vi "Update Bind Method Constants.vi"(7 "RPC Method Parameters":T1, 8 "error in (no error)":errorcluster, 10 "RPC Method Name":string, 11 "VI in":refnum<vi>) -> (0 "error out":errorcluster, 3 "VI out":refnum<vi>)   [LabVIEW 2019, in "gRPC Template Creation Utility.lvlib"]
uses:
  gRPC Template Creation Utility.lvlib
  TypeDefs/RPC Method Parameters.ctl
  <vilib>/Utility/traverseref.llb/TRef TravTarget.ctl
  <vilib>/Utility/traverseref.llb/VI Scripting - Traverse.lvlib
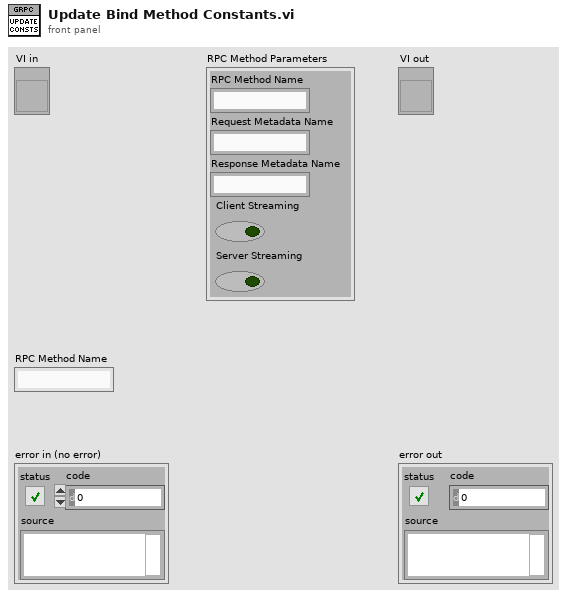
[diagram p1: front panel]
types:
  T1 = typedef "gRPC Template Creation Utility.lvlib/RPC Method Parameters.ctl" = cluster{"RPC Method Name":string, "Request Metadata Name":string, "Response Metadata Name":string, "Client Streaming":bool, "Server Streaming":bool}
  T2 = typedef "TRef TravTarget.ctl" = enum16{"FP", "BD", "Other"}
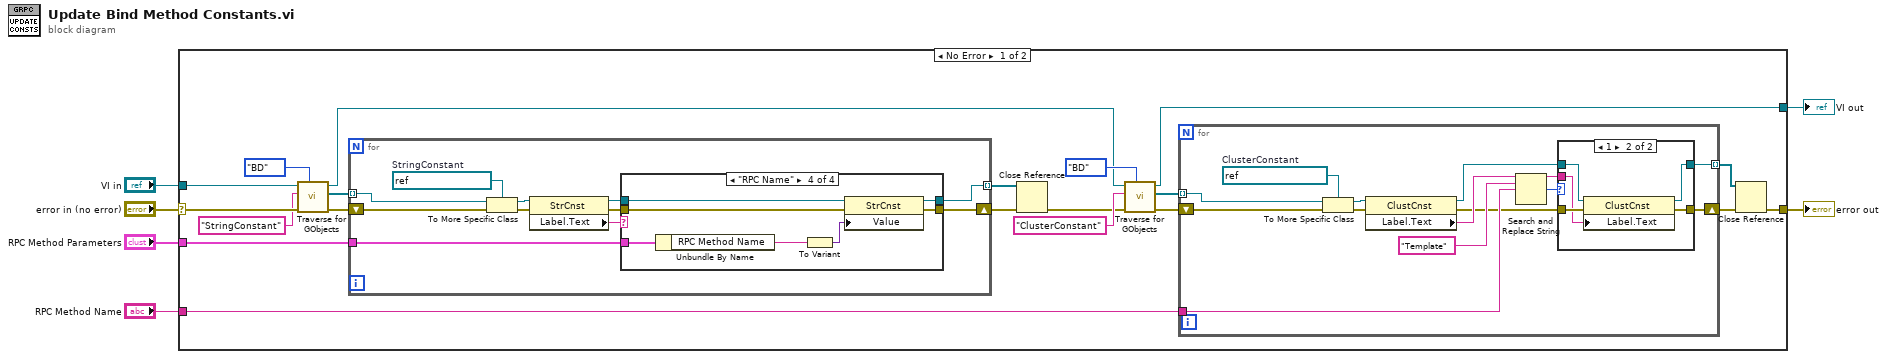
[diagram p0: block diagram]
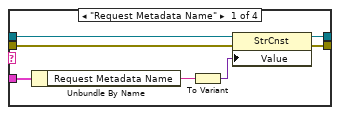
[diagram p3: hidden frame]
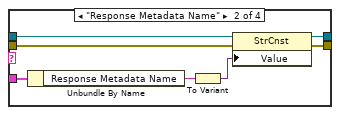
[diagram p4: hidden frame]
diagram:
  n1 = case shown="No Error" "error in (no error)" {
    selector: "error in (no error)" -> [w25 w83]
    tunnel: [w26 w83] -> w6
    tunnel: "VI in" -> [w24 w82]
    tunnel: "RPC Method Name" -> [w23 _]
    tunnel: [w7 w82] -> w2
    tunnel: "RPC Method Parameters" -> [w22 _]
    frame No Error {
      n2 = call <vilib>:"Traverse for GObjects.vi"("Traverse Target"=TRef_TravTarget."BD", "error in (no error)"=w25, "Class Name"="StringConstant", "VI Refnum"=w24) -> ("error out"=w19:errorcluster, "References"=w15:refnum<vi>[], "dup VI Refnum"=w8:refnum<vi>)  [unwired: 4 in, 1 out]
      n3 = for {
        tunnel: w15 -> [w57] mode=indexing
        shift-right: [w49] -> w16
        shift-left: w19 -> [w56]
        tunnel: w22 -> [w52]
        tunnel: [w48] -> w14 mode=indexing
        w58 = refnum<vi> refnum  # StringConstant
        n4 = To More Specific Class(target class=w58, reference=w57, error in=w56) -> (specific class reference=w55:refnum<vi>, error out=w54:errorcluster)
        n5 = property class="StrCnst"(reference=w55, error in=w54) -> (reference out=w51:refnum<vi>, error out=w50:errorcluster, "Label.Text"=w53:string)
        n6 = case shown="\"RPC Name\"" w53 {
          tunnel: w52 -> [w60 w70 _ w81]
          tunnel: w51 -> [w62 w68 w73 w80]
          tunnel: w50 -> [w63 w69 w74 w77]
          tunnel: [w61 w67 w74 w76] -> w49
          tunnel: [w59 w66 w73 w75] -> w48
          frame "Request Metadata Name" {
            n7 = Unbundle By Name(w60) -> ("Request Metadata Name"=w65:string)
            n8 = To Variant(anything=w65) -> (Variant=w64:variant)
            n9 = property class="StrCnst"(reference=w62, error in=w63, "Value"=w64) -> (reference out=w59:refnum<vi>, error out=w61:errorcluster)
          }
          frame "Response Metadata Name" {
            n10 = Unbundle By Name(w70) -> ("Response Metadata Name"=w72:string)
            n11 = To Variant(anything=w72) -> (Variant=w71:variant)
            n12 = property class="StrCnst"(reference=w68, error in=w69, "Value"=w71) -> (reference out=w66:refnum<vi>, error out=w67:errorcluster)
          }
          frame "None", Default {
          }
          frame "RPC Name" {
            n13 = Unbundle By Name(w81) -> ("RPC Method Name"=w79:string)
            n14 = To Variant(anything=w79) -> (Variant=w78:variant)
            n15 = property class="StrCnst"(reference=w80, error in=w77, "Value"=w78) -> (reference out=w75:refnum<vi>, error out=w76:errorcluster)
          }
        }
      }
      n16 = Close Reference(reference=w14, error in (no error)=w16) -> (error out=w13:errorcluster)
      n17 = call <vilib>:"Traverse for GObjects.vi"("Traverse Target"=TRef_TravTarget."BD", "error in (no error)"=w13, "Class Name"="ClusterConstant", "VI Refnum"=w8) -> ("error out"=w12:errorcluster, "References"=w11:refnum<vi>[], "dup VI Refnum"=w7:refnum<vi>)  [unwired: 4 in, 1 out]
      n18 = for {
        tunnel: w11 -> [w39] mode=indexing
        shift-right: [w28] -> w10
        shift-left: w12 -> [w38]
        tunnel: w23 -> [w33]
        tunnel: [w27] -> w9 mode=indexing
        w40 = refnum<vi> refnum  # ClusterConstant
        n19 = To More Specific Class(target class=w40, reference=w39, error in=w38) -> (specific class reference=w37:refnum<vi>, error out=w36:errorcluster)
        n20 = property class="ClustCnst"(reference=w37, error in=w36) -> (reference out=w32:refnum<vi>, error out=w31:errorcluster, "Label.Text"=w34:string)
        n21 = Search and Replace String(input string=w34, search string="Template", replace string=w33) -> (result string=w29:string, number of replacements=w30:i32)  [unwired: 5 in, 2 out]
        n22 = case shown="1" w30 {
          tunnel: w32 -> [w42 w47]
          tunnel: [w42 w46] -> w27
          tunnel: [w41 w45] -> w28
          tunnel: w31 -> [w41 w44]
          tunnel: w29 -> [_ w43]
          frame 0, Default {
          }
          frame 1 {
            n23 = property class="ClustCnst"(reference=w47, error in=w44, "Label.Text"=w43) -> (reference out=w46:refnum<vi>, error out=w45:errorcluster)
          }
        }
      }
      n24 = Close Reference(reference=w9, error in (no error)=w10) -> (error out=w26:errorcluster)
    }
    frame Error {
    }
  }
  "error out" <- w6
  "VI out" <- w2
